vi "SetValueByArrayIndex.vi"(0 "VI Reference In":refnum<vi>, 2 "delimiter (>>)":string=">>", 5 "Control Path":string, 7 "Index Array":i32[](array[numeric]), 11 "Error In":errorcluster) -> (4 "VI Reference Out":refnum<vi>, 15 "Error Out":errorcluster)   [LabVIEW 2016, in "Drona.lvlib" / "ControlValue.lvlib" / "StimulusMCListbox.lvlib"]
doc: "Sets value(signaling) for the multi select multi column listbox control whose index values are specified. \n\nThe input control name is given as a string , incase of path, use delimiters inbetween the path."
uses:
  StimulusMCListbox.lvlib
  <vilib>/Utility/error.llb/Error Cluster From Error Code.vi
  <vilib>/ErrorRing/Error Ring.xnode
  Drona.lvlib
  Get/GetControlRef/GetControlRef.lvlib
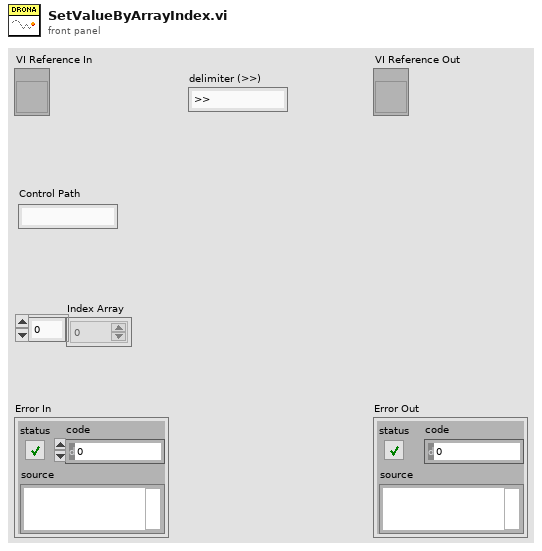
[diagram p1: front panel]
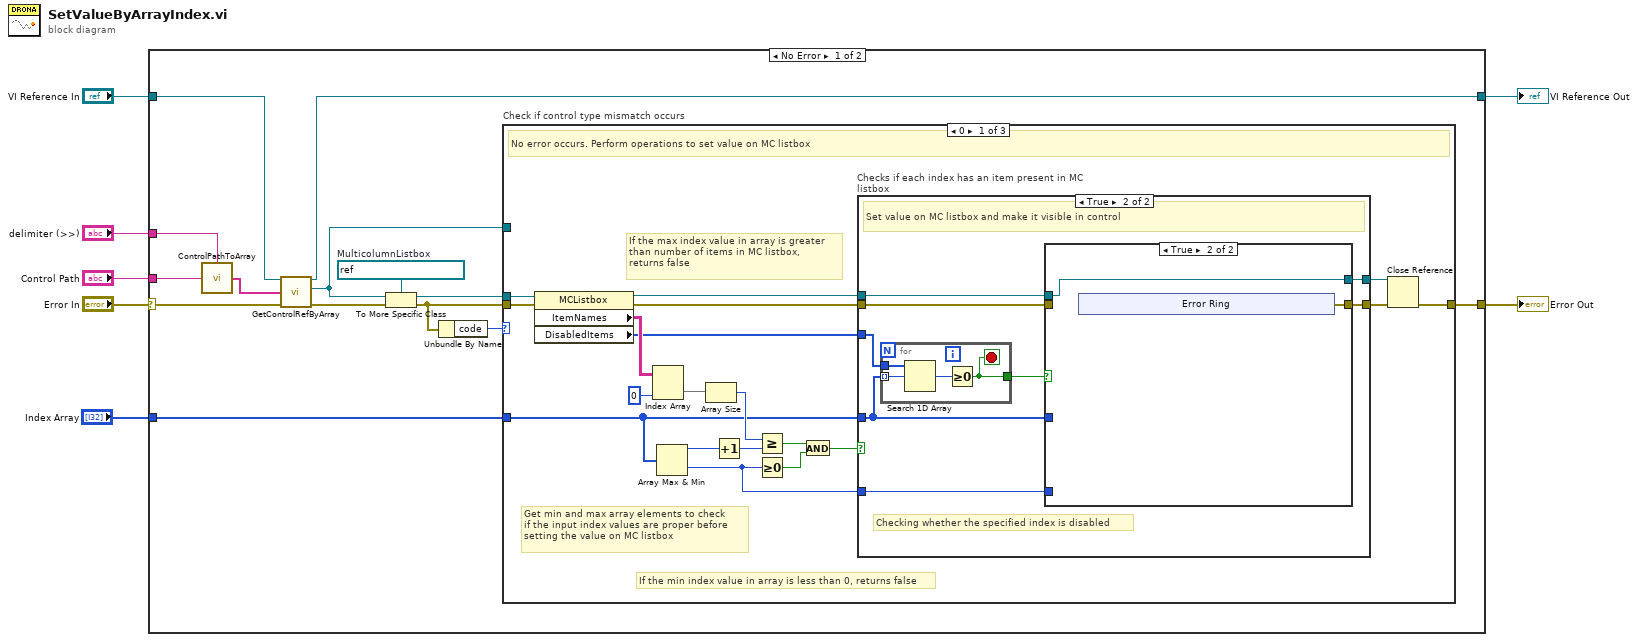
[diagram p0: block diagram]
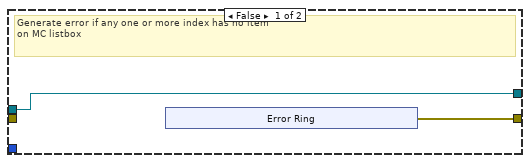
[diagram p2: hidden frame]
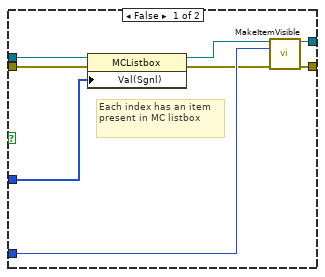
[diagram p3: hidden frame]
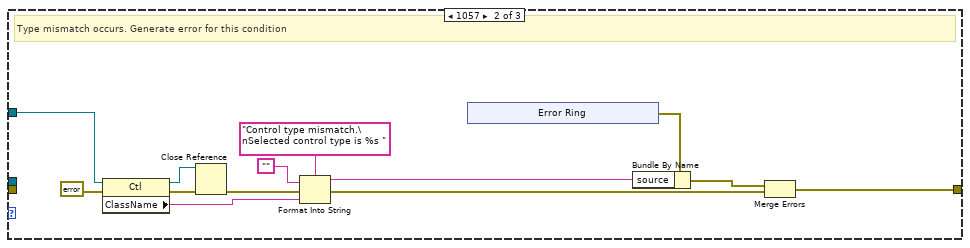
[diagram p4: hidden frame]
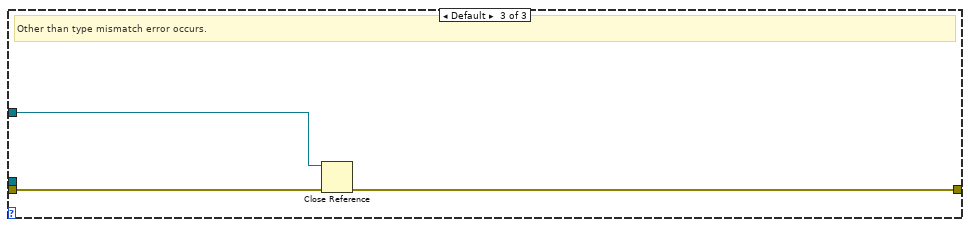
[diagram p5: hidden frame]
diagram:
  n1 = case shown="No Error" "Error In" {
    selector: "Error In" -> [w16 w97]
    tunnel: [w17 w97] -> w6
    tunnel: "VI Reference In" -> [w14 w96]
    tunnel: "Control Path" -> [w20 _]
    tunnel: "Index Array" -> [w11 _]
    tunnel: [w13 w96] -> w2
    tunnel: "delimiter (>>)" -> [w19 _]
    frame No Error {
      w21 = refnum<vi> refnum  # MulticolumnListbox
      n2 = call "ControlPathToArray.vi"("Control Name"=w20, "delimiter (>>)"=w19) -> ("Control Path"=w15:string[])
      n3 = call "GetControlRefByArray.vi"("VI Reference In"=w14, "Control Path"=w15, "error In"=w16) -> ("VI Reference Out"=w13:refnum<vi>, "Ctl Refnum"=w8:refnum<vi>, "error out"=w12:errorcluster)  [unwired: 10 in]
      n4 = To More Specific Class(target class=w21, reference=w8, error in=w12) -> (specific class reference=w18:refnum<vi>, error out=w10:errorcluster)
      n5 = Unbundle By Name(w10) -> ("code"=w9:i32)
      n6 = case "Check if control type mismatch occurs" shown="0" w9 {
        tunnel: w10 -> [w40 _ w95]
        tunnel: w18 -> [w36 _ _]
        tunnel: [w32 w75 w94] -> w17
        tunnel: w11 -> [w27 _ _]
        tunnel: w8 -> [_ w76 w93]
        frame 0 {
          # "If the min index value in array is less than 0, returns false"
          # "If the max index value in array is greater \nthan number of items in MC listbox, \nreturns false"
          # "Get min and max array elements to check \nif the input index values are proper before \nsetting the value on MC listbox"
          # "No error occurs. Perform operations to set value on MC listbox"
          n7 = property class="MCListbox"(reference=w36, error in=w40) -> (reference out=w35:refnum<vi>, error out=w37:errorcluster, "ItemNames"=w25:string[][], "DisabledItems"=w22:i32[])
          n8 = Index Array(array=w25, index (col)=0 ("disabled index (col)")) -> (element=w23:string[])  [unwired: 1 in]
          n9 = Array Max & Min(array=w27) -> (max value=w31:i32, min value=w29:i32)  [unwired: 2 out]
          n10 = Array Size(array=w23) -> (size(s)=w34:i32)
          n11 = Increment(x=w31) -> (x+1=w30:i32)
          n12 = Greater Or Equal?(x=w34, y=w30) -> (x >= y?=w28:bool)
          n13 = Greater Or Equal To 0?(x=w29) -> (x >= 0?=w26:bool)
          n14 = And(x=w28, y=w26) -> (x .and. y?=w33:bool)
          n15 = case "Checks if each index has an item present in MC listbox" shown="True" w33 {
            tunnel: [w41 w55] -> w39
            tunnel: [w42 w54] -> w38
            tunnel: w29 -> [_ w53]
            tunnel: w37 -> [_ w52]
            tunnel: w35 -> [w42 w51]
            tunnel: w27 -> [_ w50]
            tunnel: w22 -> [_ w49]
            frame False {
              # "Generate error if any one or more index has no item \non MC listbox"
              n16 = xnode "Error Ring"() -> ("error out"=w41:errorcluster)
            }
            frame True {
              # "Checking whether the specified index is disabled"
              # "Set value on MC listbox and make it visible in control"
              n17 = for {
                tunnel: w50 -> [w58] mode=indexing
                tunnel: w49 -> [w59]
                tunnel: [w56] -> w48
                stop <- w56 stop-if-true
                n18 = Search 1D Array(1D array=w59, element=w58) -> (index of element=w57:i32)  [unwired: 1 in]
                n19 = Greater Or Equal To 0?(x=w57) -> (x >= 0?=w56:bool)
              }
              n20 = case shown="True" w48 {
                tunnel: [w67 w68] -> w55
                tunnel: [w66 w69] -> w54
                tunnel: w53 -> [w65 _]
                tunnel: w52 -> [w64 _]
                tunnel: w51 -> [w62 w69]
                tunnel: w50 -> [w61 _]
                frame False {
                  # "Each index has an item present in MC listbox"
                  n21 = property class="MCListbox"(reference=w62, error in=w64, "Val(Sgnl)"=w61) -> (reference out=w60:refnum<vi>, error out=w63:errorcluster)
                  n22 = call "MakeItemVisible.vi"("MC ListBox Ref In"=w60, "Item Index"=w65, "Error In"=w63) -> ("MC ListBox Ref Out"=w66:refnum<vi>, "Error Out"=w67:errorcluster)  [unwired: 11 in]
                }
                frame True {
                  n23 = xnode "Error Ring"() -> ("error out"=w68:errorcluster)
                }
              }
            }
          }
          n24 = Close Reference(reference=w38, error in (no error)=w39) -> (error out=w32:errorcluster)
        }
        frame 1057 {
          # "Type mismatch occurs. Generate error for this condition"
          n25 = property class="Ctl"(reference=w76, error in=errorcluster {"status"=FALSE, "code"=0, "source"=""} ("error out")) -> (reference out=w77:refnum<vi>, error out=w87:errorcluster, "ClassName"=w84:string)
          n26 = Close Reference(reference=w77, error in (no error)=w87) -> (error out=w78:errorcluster)
          n27 = Format Into String(format string="Control type mismatch.\nSelected control type is %s ", initial string="", error in=w78, w84) -> (resulting string=w81:string, error out=w79:errorcluster)
          n28 = xnode "Error Ring"() -> ("error out"=w82:errorcluster)
          n29 = Bundle By Name(cluster=w82, "source"=w81) -> (w80:errorcluster)
          n30 = Merge Errors(w80, w79) -> (w75:errorcluster)
        }
        frame Default {
          # "Other than type mismatch error occurs."
          n31 = Close Reference(reference=w93, error in (no error)=w95) -> (error out=w94:errorcluster)
        }
      }
    }
    frame Error {
    }
  }
  "Error Out" <- w6
  "VI Reference Out" <- w2
